vi "Menu Action.vi"(8 "error in (no error)":errorcluster caption="错误输入（无错误）", 10 "项标识符":string, 11 "Data Viewer 输入":refnum<class "Data Viewer.lvclass">) -> (0 "error out":errorcluster caption="错误输出", 3 "Data Viewer 输出":refnum<class "Data Viewer.lvclass">)   [LabVIEW 2020, in "Data Viewer.lvlib" / "Data Viewer.lvclass"]
uses:
  Data Viewer.lvclass
  Data Viewer.lvclass/Data Viewer.ctl
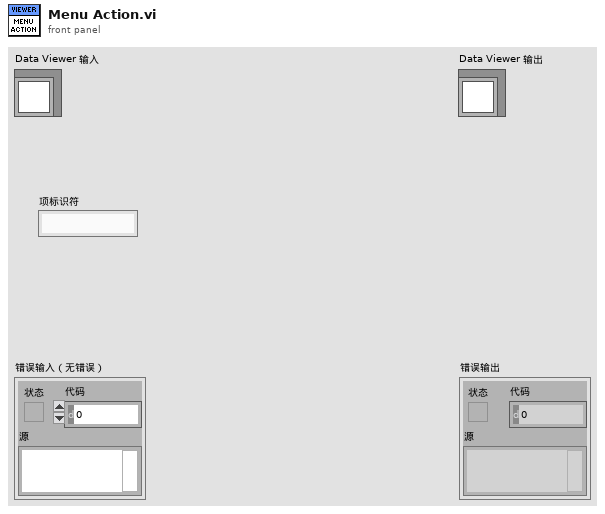
[diagram p1: front panel]
types:
  T1 = typedef "imagedata.ctl" = cluster{"image type":i32, "image depth":i32, "image":u8[], "mask":u8[], "colors":u32[], "Rectangle":cluster{"left":i16, "top":i16, "right":i16, "bottom":i16}}
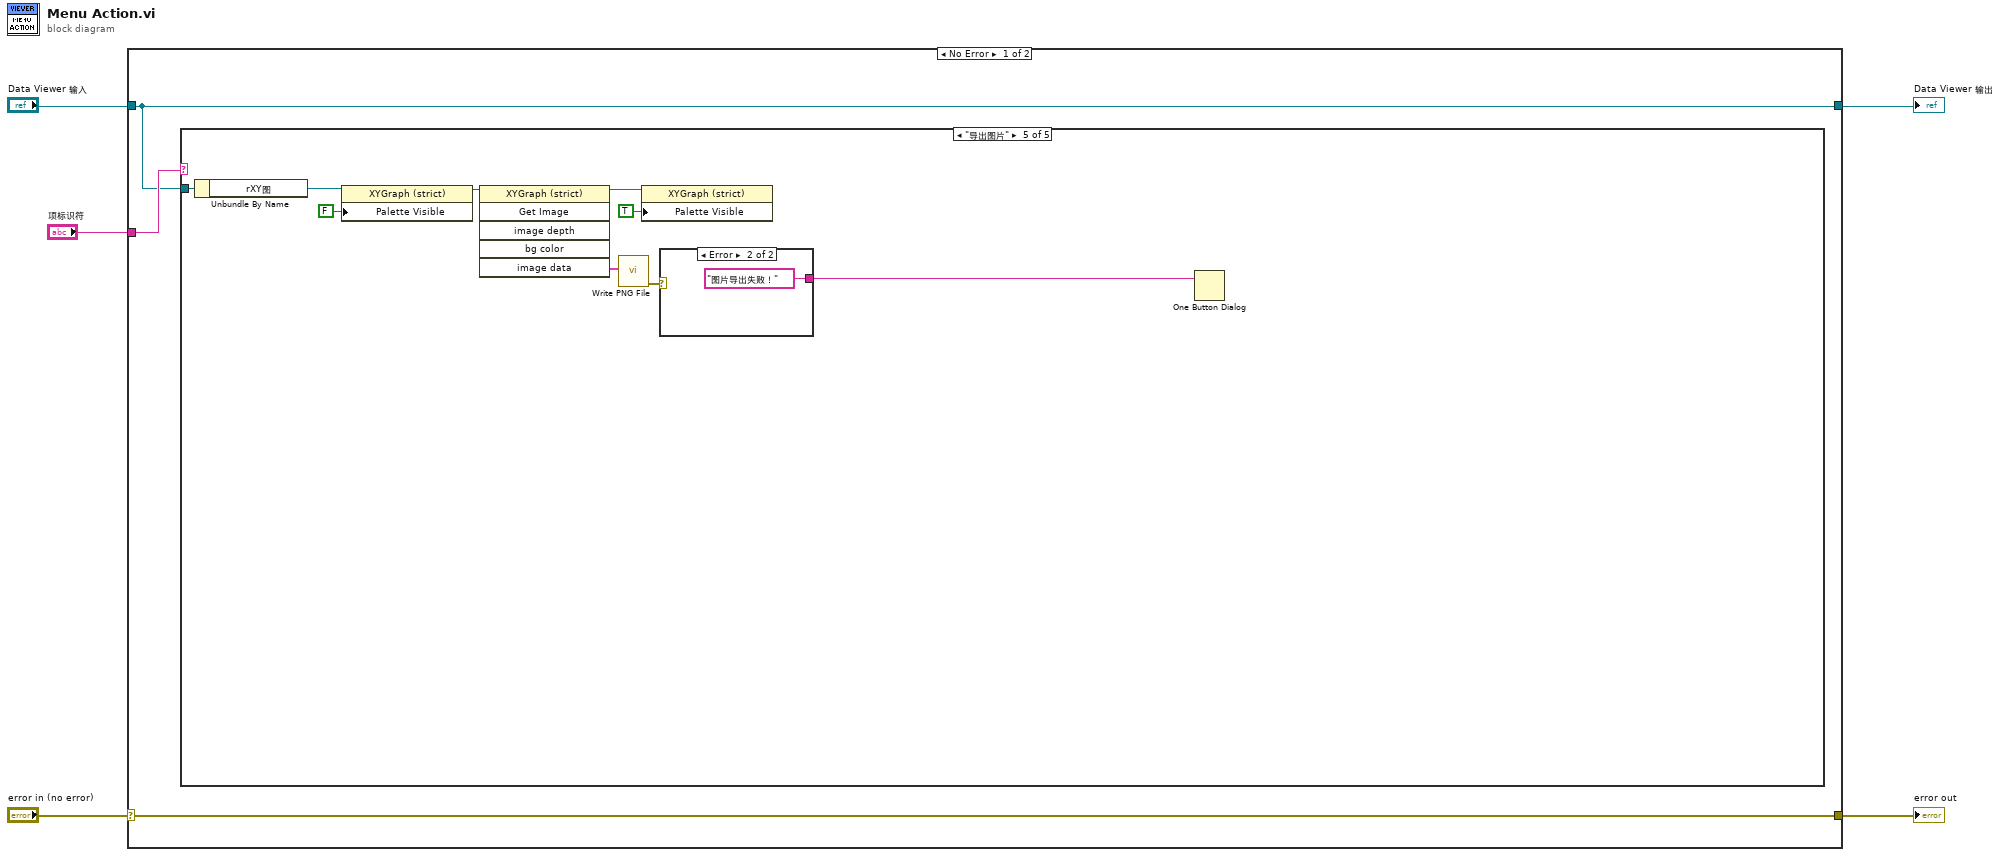
[diagram p0: block diagram]
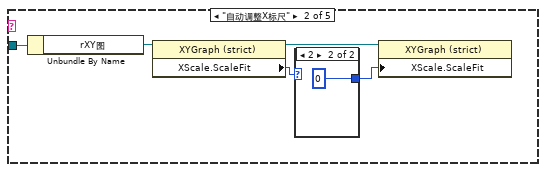
[diagram p3: hidden frame]
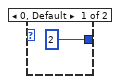
[diagram p4: hidden frame]
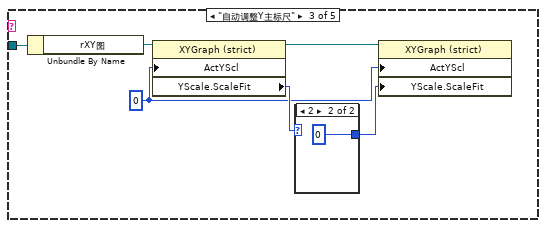
[diagram p5: hidden frame]
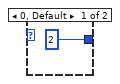
[diagram p6: hidden frame]
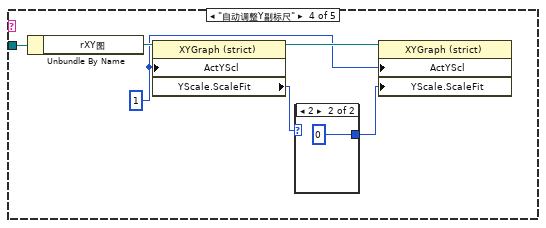
[diagram p7: hidden frame]
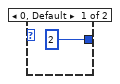
[diagram p8: hidden frame]
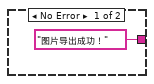
[diagram p9: hidden frame]
diagram:
  n1 = case shown="No Error" "error in (no error)" {
    selector: "error in (no error)" -> [w8 w44]
    tunnel: [w8 w44] -> w4
    tunnel: [w6 w43] -> w2
    tunnel: "Data Viewer 输入" -> [w6 w43]
    tunnel: "项标识符" -> [w7 _]
    frame No Error {
      n2 = case shown="\"导出图片\"" w7 {
        tunnel: w6 -> [_ w10 w20 w28 w37]
        frame "假", Default {
        }
        frame "自动调整X标尺" {
          n3 = Unbundle By Name(w10) -> ("rXY图"=w9:refnum<vi>)
          n4 = property class="XYGraph (strict)"(reference=w9) -> (reference out=w12:refnum<vi>, "XScale.ScaleFit"=w11:u8)  [unwired: 1 in, 1 out]
          n5 = case shown="2" w11 {
            tunnel: [u8 2 ("X标尺.标尺调节") u8 0 ("X标尺.标尺调节")] -> w13
            frame 0, Default {
            }
            frame 2 {
            }
          }
          n6 = property class="XYGraph (strict)"(reference=w12, "XScale.ScaleFit"=w13) -> ()  [unwired: 1 in, 2 out]
        }
        frame "自动调整Y主标尺" {
          w16 = 0 ("活动Y标尺")
          n7 = Unbundle By Name(w20) -> ("rXY图"=w19:refnum<vi>)
          n8 = property class="XYGraph (strict)"(reference=w19, "ActYScl"=w16) -> (reference out=w21:refnum<vi>, "YScale.ScaleFit"=w18:u8)  [unwired: 1 in, 1 out]
          n9 = case shown="2" w18 {
            tunnel: [u8 2 ("X标尺.标尺调节") u8 0 ("X标尺.标尺调节")] -> w17
            frame 0, Default {
            }
            frame 2 {
            }
          }
          n10 = property class="XYGraph (strict)"(reference=w21, "ActYScl"=w16, "YScale.ScaleFit"=w17) -> ()  [unwired: 1 in, 2 out]
        }
        frame "自动调整Y副标尺" {
          w24 = 1 ("活动Y标尺")
          n11 = Unbundle By Name(w28) -> ("rXY图"=w27:refnum<vi>)
          n12 = property class="XYGraph (strict)"(reference=w27, "ActYScl"=w24) -> (reference out=w29:refnum<vi>, "YScale.ScaleFit"=w26:u8)  [unwired: 1 in, 1 out]
          n13 = case shown="2" w26 {
            tunnel: [u8 2 ("X标尺.标尺调节") u8 0 ("X标尺.标尺调节")] -> w25
            frame 0, Default {
            }
            frame 2 {
            }
          }
          n14 = property class="XYGraph (strict)"(reference=w29, "ActYScl"=w24, "YScale.ScaleFit"=w25) -> ()  [unwired: 1 in, 2 out]
        }
        frame "导出图片" {
          n15 = Unbundle By Name(w37) -> ("rXY图"=w36:refnum<vi>)
          n16 = property class="XYGraph (strict)"(reference=w36, "Palette Visible"=FALSE ("选板:可见")) -> (reference out=w34:refnum<vi>)  [unwired: 1 in, 1 out]
          n17 = invoke class="XYGraph (strict)" method="Get Image"(reference=w34) -> (reference out=w32:refnum<vi>, "image data"=w40:T1)  [unwired: 5 in, 4 out]
          n18 = call <vilib>:"Write PNG File.vi"("image data"=w40) -> ("error out"=w39:errorcluster)  [unwired: 9 in, 1 out]
          n19 = property class="XYGraph (strict)"(reference=w32, "Palette Visible"=TRUE ("选板:可见")) -> ()  [unwired: 1 in, 2 out]
          n20 = case shown="Error" w39 {
            tunnel: ["图片导出成功！" "图片导出失败！"] -> w38
            frame No Error {
            }
            frame Error {
            }
          }
          n21 = One Button Dialog(message=w38) -> ()  [unwired: 1 in, 1 out]
        }
      }
    }
    frame Error {
    }
  }
  "error out" <- w4
  "Data Viewer 输出" <- w2
